vi "load tags from cvt1.vi"(10 "vi path":path, 11 "engine ref":refnum<data-value>) -> (2 "load attempted":bool)   [LabVIEW 2013, in "PL Framework Configuration Tool.lvlib" / "EngineTags.lvclass"]
uses:
  EngineTags.lvclass
  Engine Parent/Engine Parent Editor Node.lvclass
  <vilib>/NI/Module Execution Interface/Engine Configuration/engine configuration.lvclass
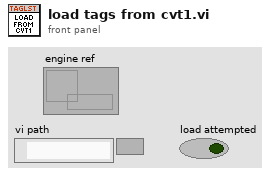
[diagram p1: front panel]
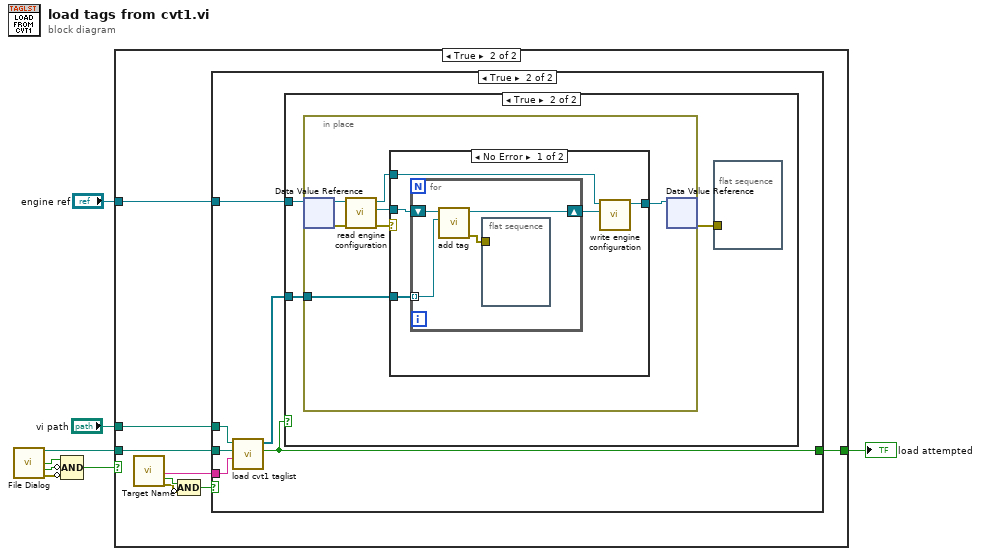
[diagram p0: block diagram]
diagram:
  n1 = call "File Dialog"() -> ("selected path"=w5:path, "exists"=w4:bool, "cancelled"=w3:bool, "error out"=w2:errorcluster)  [unwired: 12 in]
  n2 = Compound Arithmetic op=AND(w4, invert w3, invert w2) -> (w6:bool)
  n3 = case shown="True" w6 {
    tunnel: w5 -> [_ w16]
    tunnel: [_ w11] -> w8
    tunnel: "vi path" -> [_ w10]
    tunnel: "engine ref" -> [_ w9]
    frame False {
    }
    frame True {
      n4 = call "Target Name"() -> ("Target Name"=w15:string, "OK"=w14:bool, "error out"=w13:errorcluster)  [unwired: 17 in]
      n5 = Compound Arithmetic op=AND(w14, invert w13) -> (w12:bool)
      n6 = case shown="True" w12 {
        tunnel: w16 -> [_ w21]
        tunnel: w15 -> [_ w20]
        tunnel: [_ w19] -> w11
        tunnel: w10 -> [_ w18]
        tunnel: w9 -> [_ w17]
        frame False {
        }
        frame True {
          n7 = call "load cvt1 taglist.vi"("target name"=w20, "cfg file path"=w21, "vi path"=w18) -> ("ok?"=w19:bool, "tags"=w22:refnum<class "tag descriptor.lvclass">[])  [unwired: 7 in]
          n8 = case shown="True" w19 {
            tunnel: w22 -> [_ w24]
            tunnel: w17 -> [_ w23]
            frame False {
            }
            frame True {
              n9 = in-place {
                in-place-border: w24 -> [w32]
                n10 = in-place-dvr #1(w23) -> (w30:refnum<class "Engine Parent Editor Node.lvclass">, w31:errorcluster)
                n11 = call "read engine configuration.vi"("error in"=w31, "Engine Parent Editor Node in"=w30) -> ("error out"=w27:errorcluster, "engine configuration"=w26:refnum<class "engine configuration.lvclass">, "Engine Parent Editor Node out"=w29:refnum<class "Engine Parent Editor Node.lvclass">)  [unwired: 7 in]
                n12 = case shown="No Error" w27 {
                  tunnel: w32 -> [w37 _]
                  tunnel: w29 -> [w35 w42]
                  tunnel: [w34 w42] -> w28
                  tunnel: w26 -> [w33 _]
                  frame No Error {
                    n13 = for {
                      shift-right: [w41] -> w36
                      shift-left: w33 -> [w40]
                      tunnel: w37 -> [w39] mode=indexing
                      n14 = call <vilib>:"add tag.vi"("tag descriptor"=w39, "engine configuration in"=w40) -> ("error out"=w38:errorcluster, "engine configuration out"=w41:refnum<class "engine configuration.lvclass">)  [unwired: 8 in]
                      n15 = flat-sequence {
                        tunnel: w38 -> [_]
                        frame #0 {
                        }
                      }
                    }
                    n16 = call "write engine configuration.vi"("engine configuration"=w36, "Engine Parent Editor Node in"=w35) -> ("Engine Parent Editor Node out"=w34:refnum<class "Engine Parent Editor Node.lvclass">)  [unwired: 8 in, 1 out]
                  }
                  frame Error {
                  }
                }
                n17 = in-place-dvr #1(w28) -> (w25:errorcluster)  [unwired: 1 out]
              }
              n18 = flat-sequence {
                tunnel: w25 -> [_]
                frame #0 {
                }
              }
            }
          }
        }
      }
    }
  }
  "load attempted" <- w8
